vi "Day 20-Add Padding.vi"(10 "Padding Value":bool, 11 "Array in":bool[][](array[boolean])) -> (3 "Array out":bool[][](array[boolean]))   [LabVIEW 2021]
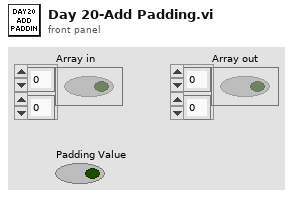
[diagram p1: front panel]
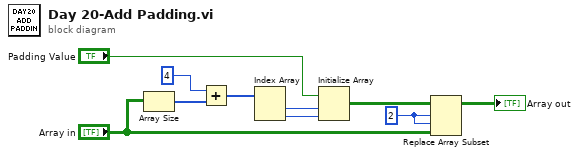
[diagram p0: block diagram]
diagram:
  w3 = 2 ("index (row)")
  n1 = Array Size(array="Array in") -> (size(s)=w8:i32[])
  n2 = Add(x=4, y=w8) -> (x+y=w6:i32[])
  n3 = Index Array(array=w6) -> (element #1=w5:i32, element #2=w4:i32)  [unwired: 2 in]
  n4 = Initialize Array("Padding Value", w5, w4) -> (w2:bool[][])
  n5 = Replace Array Subset(array=w2, new element="Array in", index (row)=w3, index (col)=w3) -> (→"Array out":bool[][])
